vi "Signals.Scale.EU.vi"(4 "Buffer?":bool, 5 "Lookup":variant, 6 "Type":T1, 7 "Reads Ref":T2, 8 "error in (no error)":errorcluster, 10 "Unscaled Data":u8[](array[numeric]), 11 "ID":u32) -> (0 "error out":errorcluster)   [LabVIEW 2024, in "Diagnostics Addon Engine.lvlib"]
uses:
  Diagnostics Addon Engine.lvlib
  <vilib>/NI/NIVS Inline Async API/_Data Access Engine/Data Access Engine/Types/Write.DVR.ctl
  <vilib>/NI/NIVS Inline Async API/_Data Access Engine/Access Type Classes/Write/Write.lvclass
  Addon Shared/Types/Type.ctl
  Addon Shared/Types/Frame.Lookup.Info.ctl
  <vilib>/xnet/xnet.llb/XNET Frame CAN.ctl
  <vilib>/xnet/xnet.llb/XNET Frame Type CAN.ctl
  <vilib>/NI/NIVS Inline Async API/_Data Access Engine/Access Type Classes/Write/Write.lvclass/Write.ctl
  <vilib>/NI/NIVS Inline Async API/_Data Access Engine/Data Access Engine/Methods/Write.Data.Buffer.vi
  <vilib>/NI/NIVS Inline Async API/_Data Access Engine/Data Access Engine/Methods/Write.Data.vi
  <vilib>/NI/NIVS Inline Async API/_Data Access Engine/Access Type Classes/Write/Write.Buffer.vi
  <vilib>/NI/NIVS Inline Async API/_Data Access Engine/Access Type Classes/Write/Write.ProcessData.vi
  <vilib>/NI/NIVS Inline Async API/_Data Access Engine/Access Type Classes/Write/Write.Commit.vi
  Addon Shared/SubVIs/Constants.vi
  <vilib>/xnet/xnet.llb/XNET Convert (Frame CAN to Signal).vi
  Addon Shared/Diagnostics Addon Shared.lvlib
  <vilib>/NI/NIVS Inline Async API/_Data Access Engine/Data Access Engine/Data Access Engine.lvclass
  <vilib>/Utility/SystemLogging/NI_SystemLogging.lvlib
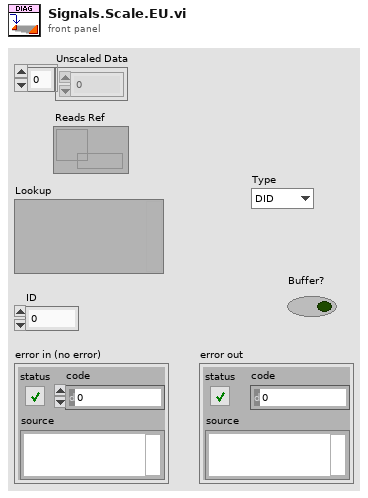
[diagram p1: front panel]
types:
  T1 = typedef "Diagnostics Addon Shared.lvlib/Type.ctl" = enum16{"DID", "CDID", "PID", "CPID", "Read Memory", "Write Memory", "IO Control", "Routine Start", "Routine Request", "Routine Stop", "User Defined", "DTC Control", "Clear DTCs", "Read DTCs", "Start DTCs", "DTC Change Count", "Tester Present", "Unlock ECU", "Reset ECU", "Diag Session Control", "Communication Control", "DPID Control", "Poll Control", "Diag Comm Port Control"}
  T2 = typedef "Data Access Engine.lvlib/Data Access Engine.lvclass/Write.DVR.ctl" = refnum<data-value>
  T3 = enum16{"Output/Write", "Input/Read", "Input/ReadWrite"}
  T4 = typedef "Diagnostics Addon Shared.lvlib/Frame.Lookup.Info.ctl" = cluster{"Offset":i32, "Length":i32, "ByteLength":u16}
  T5 = typedef "XNET Frame CAN.ctl" = cluster{"timestamp":timestamp, "payload":u8[], "identifier":u32, "type":T6, "extended?":bool, "echo?":bool}
  T6 = typedef "XNET Frame Type CAN.ctl" = u8
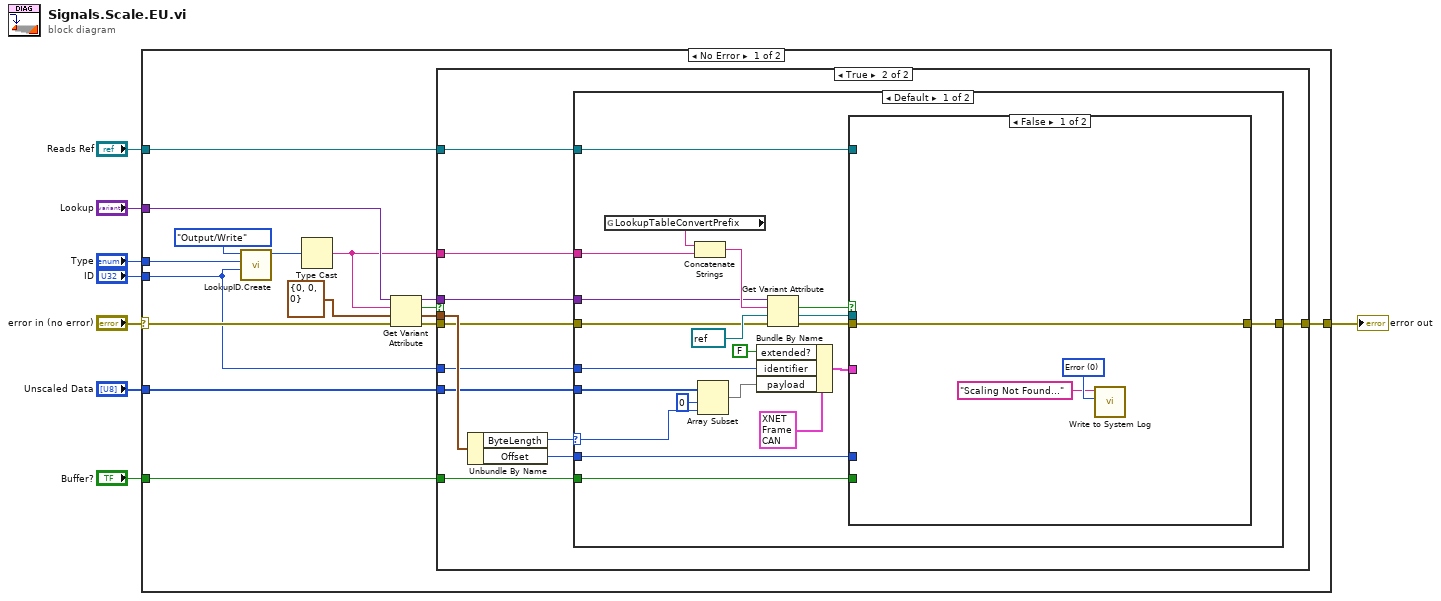
[diagram p0: block diagram]
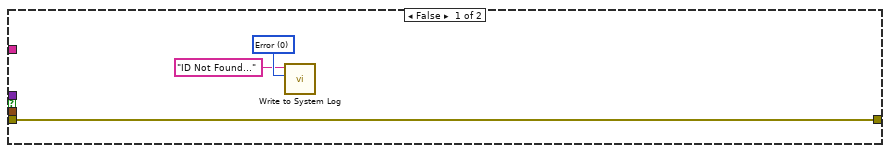
[diagram p2: hidden frame]
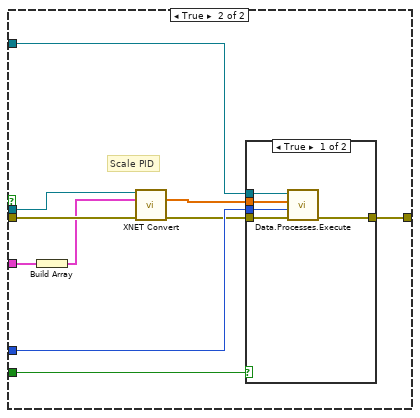
[diagram p3: hidden frame]
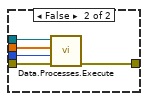
[diagram p4: hidden frame]
diagram:
  n1 = case shown="No Error" "error in (no error)" {
    selector: "error in (no error)" -> [w22 w84]
    tunnel: "Reads Ref" -> [w24 _]
    tunnel: "Lookup" -> [w21 _]
    tunnel: [w23 w84] -> w6
    tunnel: "Unscaled Data" -> [w15 _]
    tunnel: "ID" -> [w13 _]
    tunnel: "Type" -> [w14 _]
    tunnel: "Buffer?" -> [w16 _]
    frame No Error {
      n2 = call "LookupID.Create.vi"("Serivce ID"=w13, "Service Type"=w14, "Direction"=T3."Output/Write") -> ("Result"=w11:u64)  [unwired: 8 in]
      n3 = Type Cast(x=w11) -> (*(type *) &x=w18:string)  [unwired: 1 in]
      n4 = Get Variant Attribute(Variant=w21, name=w18, default value (empty Variant)=T4 {"Offset"=0, "Length"=0, "ByteLength"=0} ("cluster"), error in=w22) -> (duplicate Variant=w17:variant, found=w9:bool, value=w20:T4, error out=w10:errorcluster)
      n5 = case shown="True" w9 {
        tunnel: w24 -> [_ w38]
        tunnel: [w27 w37] -> w23
        tunnel: w20 -> [_ w36]
        tunnel: w18 -> [_ w35]
        tunnel: w17 -> [_ w34]
        tunnel: w16 -> [_ w33]
        tunnel: w15 -> [_ w31]
        tunnel: w13 -> [_ w30]
        tunnel: w10 -> [w27 w29]
        frame False {
          w26 = 0 items=["Error", "Warning", "Informational"] ("severity")
          n6 = call <vilib>:"Write to System Log.vi"("severity"=w26, "message"="ID Not Found..." ("Message")) -> ()  [unwired: 9 in, 1 out]
        }
        frame True {
          n7 = Unbundle By Name(w36) -> ("ByteLength"=w28:u16, "Offset"=w32:i32)
          n8 = case shown="Default" w28 {
            selector: w28 -> [w39 _]
            tunnel: w38 -> [w59 _]
            tunnel: [w58 w83] -> w37
            tunnel: w35 -> [w51 _]
            tunnel: w34 -> [w49 _]
            tunnel: w33 -> [w45 _]
            tunnel: w32 -> [w44 _]
            tunnel: w31 -> [w43 _]
            tunnel: w30 -> [w41 _]
            tunnel: w29 -> [w40 w83]
            frame Default {
              n9 = global read "Constants.vi" "LookupTableConvertPrefix"() -> (w57:string)
              n10 = Concatenate Strings(w57, w51) -> (w55:string)
              n11 = Array Subset(array=w43, index=0, length=w39) -> (w42:u8[])
              n12 = Bundle By Name(cluster=T5 {"timestamp"=timestamp(0 s since 1904-01-01), "payload"=[], "identifier"=0, "type"=0, "extended?"=FALSE, "echo?"=FALSE} ("CAN frame"), "extended?"=FALSE, "identifier"=w41, "payload"=w42) -> (w47:T5)
              n13 = Get Variant Attribute(Variant=w49, name=w55, default value (empty Variant)=refnum<k21> refnum ("DID Conversion"), error in=w40) -> (found=w52:bool, value=w53:refnum<k21>, error out=w56:errorcluster)  [unwired: 1 out]
              n14 = case shown="False" w52 {
                tunnel: w59 -> [_ w66]
                tunnel: [w62 w64] -> w58
                tunnel: w56 -> [w62 w72]
                tunnel: w53 -> [_ w71]
                tunnel: w44 -> [_ w68]
                tunnel: w47 -> [_ w70]
                tunnel: w45 -> [_ w63]
                frame False {
                  w61 = 0 items=["Error", "Warning", "Informational"] ("severity")
                  n15 = call <vilib>:"Write to System Log.vi"("severity"=w61, "message"="Scaling Not Found..." ("Message")) -> ()  [unwired: 9 in, 1 out]
                }
                frame True {
                  # "Scale PID"
                  n16 = Build Array(w70) -> (w69:T5[])
                  n17 = call-poly <vilib>:"XNET Convert.vi"("session in"=w71, "frame data"=w69, "error in (no error)"=w72) -> ("signal data"=w67:dbl[], "error out"=w65:errorcluster)  [unwired: 10 in, 1 out]
                  n18 = case shown="True" w63 {
                    tunnel: w68 -> [w77 w82]
                    tunnel: w67 -> [w76 w81]
                    tunnel: w66 -> [w75 w78]
                    tunnel: w65 -> [w74 w80]
                    tunnel: [w73 w79] -> w64
                    frame True {
                      n19 = call-poly <vilib>:"Data.Processes.Execute.vi"("error in (no error)"=w74, "Offset"=w77, "Values"=w76, "Ref"=w75) -> ("error out"=w73:errorcluster)  [unwired: 7 in]
                    }
                    frame False {
                      n20 = call-poly <vilib>:"Data.Processes.Execute.vi"("error in (no error)"=w80, "Offset"=w82, "Values"=w81, "Ref"=w78) -> ("error out"=w79:errorcluster)  [unwired: 7 in]
                    }
                  }
                }
              }
            }
            frame 0 {
            }
          }
        }
      }
    }
    frame Error {
    }
  }
  "error out" <- w6
